vi "Start Market.vi"(8 "error in":errorcluster) -> (0 "error out":errorcluster, 3 "stock names":string[](array[string]))   [LabVIEW 2020, in "Full Featured MCP Server.lvlib"]
doc: "Builds the simulated market (with half an hour of history and news) and returns the stock names. main.vi calls it once before the server starts."
uses:
  Full Featured MCP Server.lvlib
  Market/Market Mode.ctl
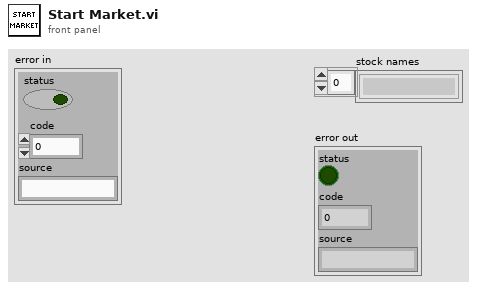
[diagram p1: front panel]
types:
  T1 = typedef "Full Featured MCP Server.lvlib/Market Mode.ctl" = enum16{"Get", "Init", "Advance", "Buy", "Sell"}
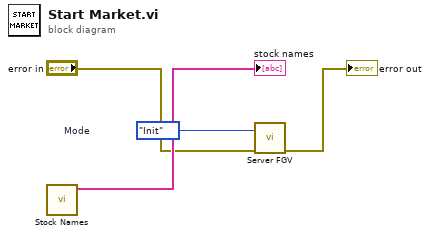
[diagram p0: block diagram]
diagram:
  w2 = Market_Mode."Init"  # Mode
  n1 = call "Stock Names.vi"() -> ("names"=→"stock names":string[])  [unwired: 11 in]
  n2 = call "Server FGV.vi"("Mode"=w2, "error in"="error in") -> ("error out"=→"error out":errorcluster)  [unwired: 7 in, 2 out]
